vi "Ejercicio3_masa_resorte.vi"() -> ()   [LabVIEW 2026]
doc: "Simulador de un sistema masa-muelle-amortiguador (Actividad EC1, Control Industrial Aplicado).\n\nModelo: m·x'' = F - D·x' - KF·x. La aceleración se calcula en un Formula Node y se integra dos veces con SubVI_Integrator.vi (método de Euler) para obtener la velocidad y la posición.\n\nEntradas: fuerza F [N], masa m [kg], constante del muelle KF [N/m] y amortiguamiento D [N/(m/s)]. Paso de integración Ts y factor de velocidad en la pestaña Time settings.\nSalidas: posición x(t) [m], gráficos de posición y fuerza, y parámetros del sistema de segundo orden K = 1/KF, z = D/(2·v(m·KF)) y w0 = v(KF/m).\n\nAutores: \nJon Ander Areizaga\nJon Fenandez\nCarlos Esparza\nManuel Jose Narvaez"
panel:
  out "Posición x [m]":dbl(graph)
  out "y [m]":dbl(slide) scale=-4.0..4.0 scale format="%.1f"
  out "Fuerza F [N]":dbl(graph)
  in  "Force\nF [N]":dbl(slide) scale=-8.0..8.0 scale format="%.1f"
  in  "Tab Control":enum32{"Time settings", "Model", "About"}(tab)
  in  "Speed_factor":dbl=5.0
  in  "Ts [s]":dbl=0.01
  in  "Spring constant\nKf":dbl(knob)=2.0 scale=1.0..10.0 scale format="%.1f"
  in  "Mass\nm":dbl(knob)=20.0 scale=0.0..40.0 scale format="%.1f"
  in  "Damping constant\nD":dbl(knob)=4.0 scale=0.0..5.0 scale format="%.1g"
  out "K [m/N]":dbl format="%.3f"
  out "z":dbl format="%#_3g"
  out "w0 [rad/s]":dbl format="%#_3g"
  in  "stop":bool
  # "SimView"
  # "Mass Spring Damper"
  # "[kg]"
  # "[N/m]"
  # "[N/(m/s)]"
  # "Transfer function from F to y:"
  # "y(s)/F(s) = K/[(s/w0)^2 + 2*z*(s/w0) + 1]"
  # "where:\n             K=1/Kf;\n             z=(D/(sqrt(m*Kf)))/2;\n             w0=sqrt(Kf/m);"
  # "GRUPO 1\nIntegrantes"
  # "Jon Ander Areizaga\nJon Fernández\nCarlos Esparza\nManuel José Narváez"
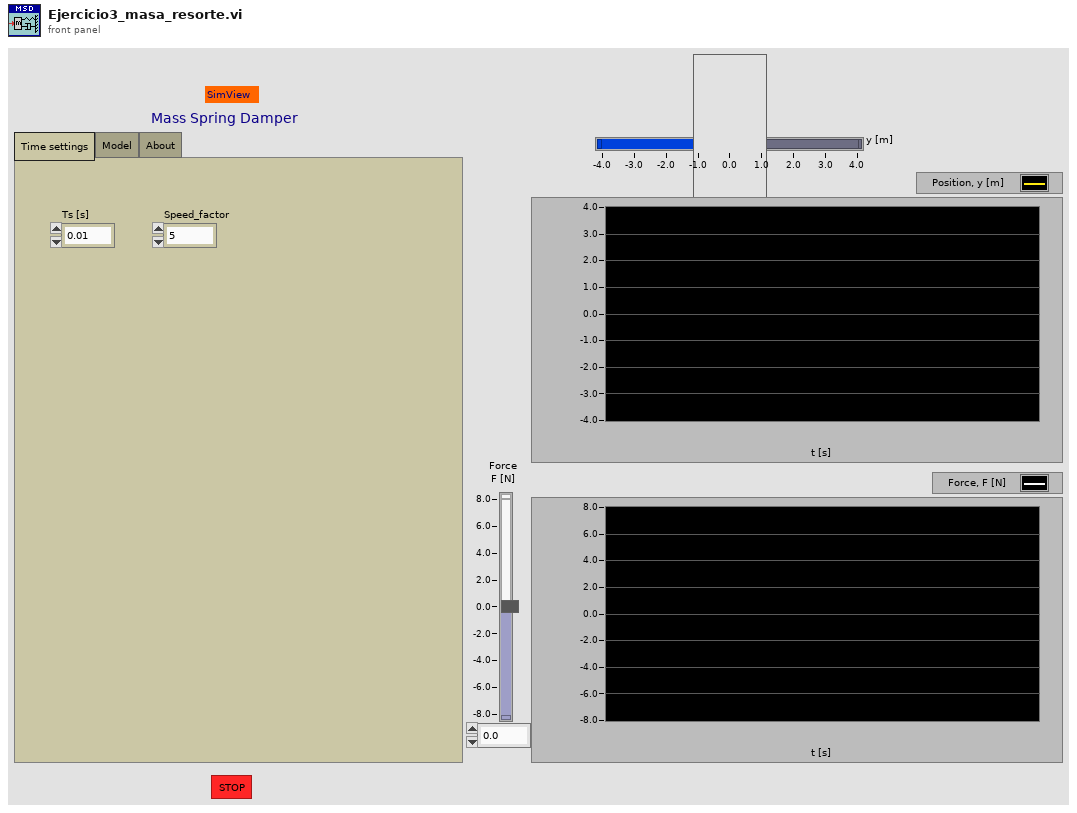
[diagram p1: front panel]
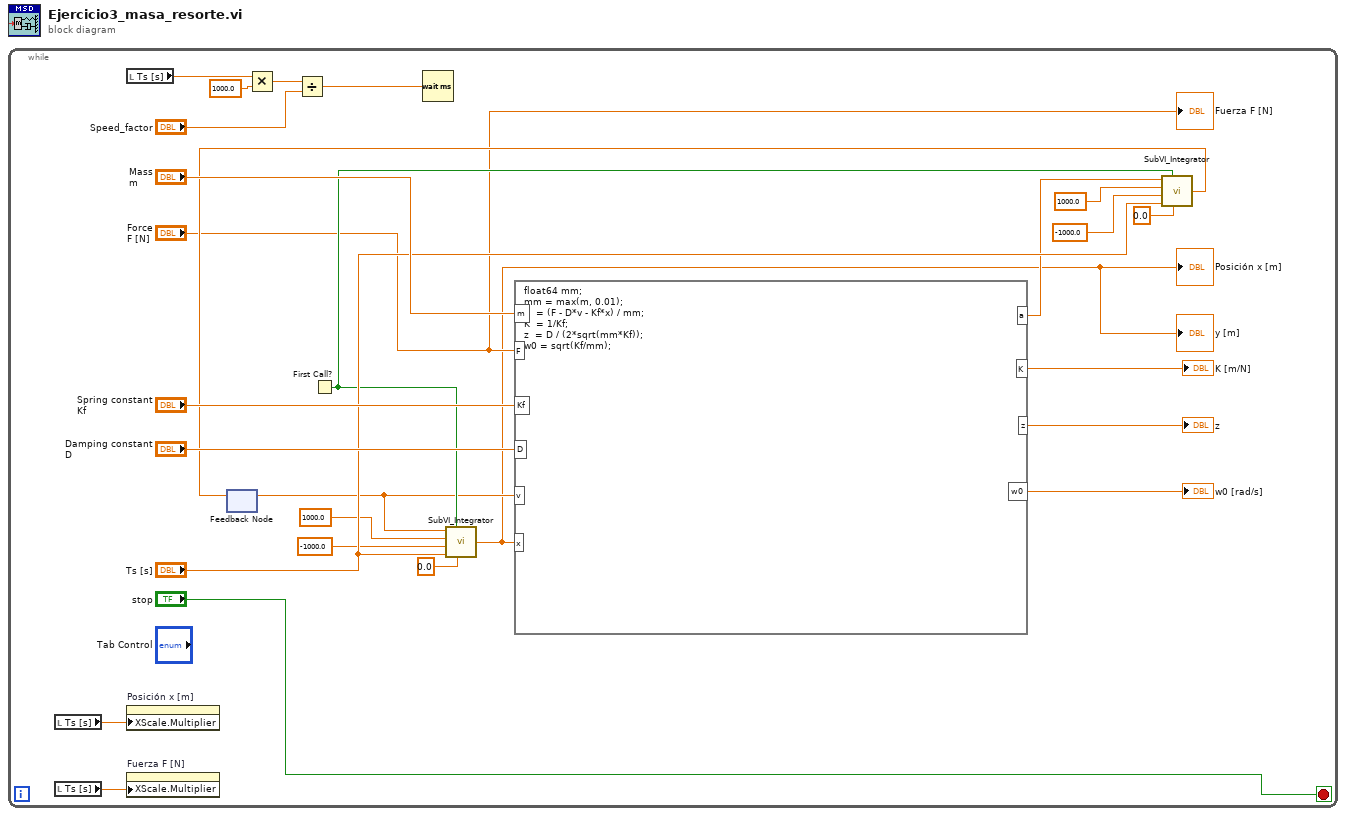
[diagram p0: block diagram]
diagram:
  n1 = while {
    stop <- "stop" stop-if-true
    n2 = local read "Ts [s]"() -> (w1:dbl)
    n3 = local read "Ts [s]"() -> (w6:dbl)
    n4 = local read "Ts [s]"() -> (w10:dbl)
    n5 = property on="Posición x [m]" class="WFChart (strict)"("XScale.Multiplier"=w1) -> ()  [unwired: 2 in, 2 out]
    n6 = property on="Fuerza F [N]" class="WFChart (strict)"("XScale.Multiplier"=w6) -> ()  [unwired: 2 in, 2 out]
    n7 = feedback #1() -> (w13:dbl)  [unwired: 1 in]
    n8 = Multiply(x=w10, y=1000.0) -> (x*y=w9:dbl)
    n9 = Divide(x=w9, y="Speed_factor") -> (x/y=w7:dbl)
    n10 = First Call?() -> (First Call?: T/F=w22:bool)
    n11 = Wait (ms)(milliseconds to wait=w7) -> ()  [unwired: 1 out]
    n12 = call "SubVI_Integrator.vi"("y_init"=0.0, "Init"=w22, "T_step [s]"="Ts [s]", "y_min"=-1000.0, "y_max"=1000.0, "u"=w13) -> ("y"=w2:dbl)
    "y [m]" <- w2
    "Posición x [m]" <- w2
    n13 = formula code="float64 mm;\nmm = max(m, 0.01);\na  = (F - D*v - Kf*x) / mm;\nK  = 1/Kf;\nz  = D / (2*sqrt(mm*Kf));\nw0 = sqrt(Kf/mm);"("m"="Mass\nm", "F"="Force\nF [N]", "Kf"="Spring constant\nKf", "D"="Damping constant\nD", "v"=w13, "x"=w2) -> ("a"=w15:dbl, "K"=→"K [m/N]":dbl, "z"=→"z":dbl, "w0"=→"w0 [rad/s]":dbl)
    n14 = call "SubVI_Integrator.vi"("y_init"=0.0, "Init"=w22, "T_step [s]"="Ts [s]", "y_min"=-1000.0, "y_max"=1000.0, "u"=w15) -> ("y"=w14:dbl)
    n15 = feedback-in #1(w14) -> ()
    "Fuerza F [N]" <- "Force\nF [N]"
  }
